vi "Split String.vi"(10 "分隔字符(;)":string=";", 11 "字符串":string) -> (2 "计数":i32, 3 "字符串数组":string[](array[string]))   [LabVIEW 2020, in "Data Viewer.lvlib"]
uses:
  Data Viewer.lvlib
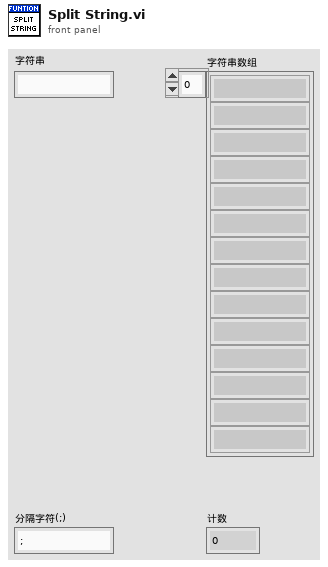
[diagram p1: front panel]
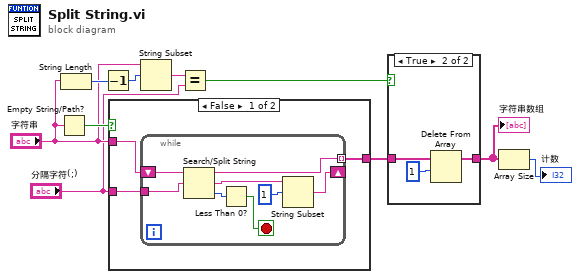
[diagram p0: block diagram]
diagram:
  n1 = Empty String/Path?(string/path="字符串") -> (empty?=w9:bool)
  n2 = String Length(string="字符串") -> (length=w8:i32)
  n3 = Decrement(x=w8) -> (x-1=w7:i32)
  n4 = case shown="False" w9 {
    tunnel: "分隔字符(;)" -> [w13 _]
    tunnel: [w12 _] -> w3
    tunnel: "字符串" -> [w11 _]
    frame False {
      n5 = while {
        shift-right: [w15] -> _
        shift-left: w11 -> [w21]
        tunnel: [w18] -> w12 mode=indexing
        tunnel: w13 -> [w14]
        stop <- w19 stop-if-true
        n6 = Search/Split String(string=w21, search string/char (-)=w14) -> (substring before match=w18:string, match + rest of string=w17:string, offset of match=w20:i32)  [unwired: 1 in]
        n7 = Less Than 0?(x=w20) -> (x < 0?=w19:bool)
        n8 = String Subset(string=w17, offset (0)=1 ("偏移量(0)")) -> (substring=w15:string)  [unwired: 1 in]
      }
    }
    frame True {
    }
  }
  n9 = String Subset(string="字符串", offset (0)=w7) -> (substring=w5:string)  [unwired: 1 in]
  n10 = Equal?(x=w5, y="分隔字符(;)") -> (x = y?=w2:bool)
  n11 = case shown="True" w2 {
    tunnel: w3 -> [w22 w25]
    tunnel: [w22 w23] -> w1
    frame False {
    }
    frame True {
      n12 = Delete From Array(array=w25, length=1 ("长度")) -> (array with subset deleted=w23:string[])  [unwired: 1 in, 1 out]
    }
  }
  "字符串数组" <- w1
  n13 = Array Size(array=w1) -> (size(s)=→"计数":i32)
